vi "JocAcabatEntregableAmbSubVis.vi"() -> ()   [LabVIEW 2023]
uses:
  <vilib>/MakerHub/LINX/Private/Local IO/LinxAnalogRead.vi
  <vilib>/MakerHub/LINX/Public/Utilities/Check Channel.vi
  <vilib>/MakerHub/LINX/Private/Utilties/Generate Error.vi
  <vilib>/MakerHub/LINX/Private/Device/Peripheral/Analog/Analog Read.vi
  <vilib>/MakerHub/LINX/Public/Utilities/Open Serial.vi
  <vilib>/MakerHub/LINX/LMH-LINX.lvlib
panel:
  out "?":string
  out "?":string="Benvingut a la jungla! El teu objectiu és sobreviure! Per aconseguir-ho, has de caçar les preses (punts verds) i fugir dels depredadors (punts vermells). Alerta, a mida que vagis avançant en el joc, aniràn apreixent més preses i depredadors. Per sort, si t'estàs a punt de quedar sense vides, apareixerà un quadrat groc, si l'atrapes, et proporcionarà una vida extra. També has de tenir en compte que tens 40 s per atrapar les preses, si tardes més, et moriràs de gana... Abans que passi però, apareixerà un diamant groc. Atrapa'l i tindràs una mica més de temps per caçar. Bona sort! "
  out "Nivell:":i32
  in  "base path":path
  in  "Serial Port":refnum<visa-resource-name>="N/A"
  out "Tablero":cluster{dbl[], dbl[]}[](graph)
  out "Vides":i32
  out "Preses capturades":i32
  out "Temps sense \nmenjar (ms)":u32
  in  "?":bool
  out "ms totals":u32
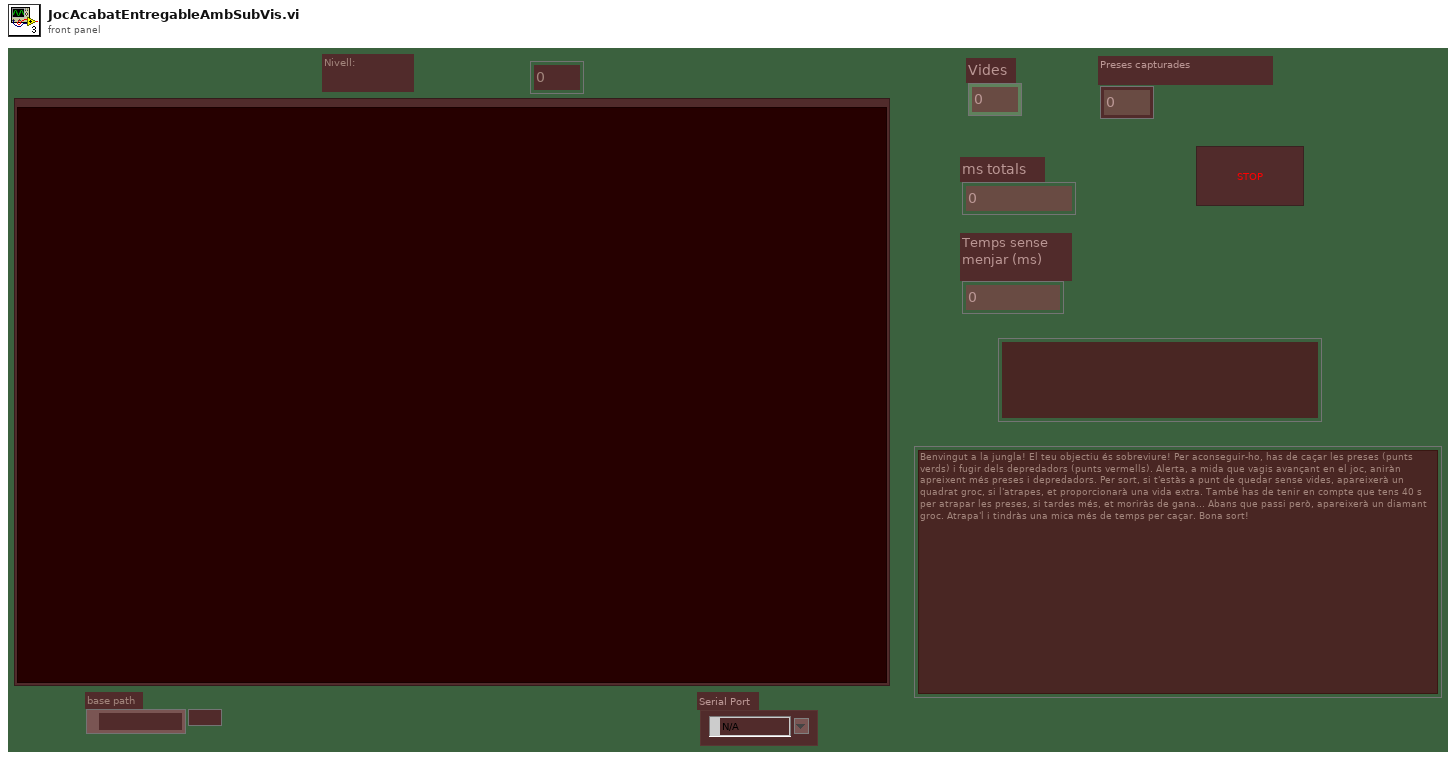
[diagram p1: front panel]
types:
  T1 = enum16{"open", "replace", "create", "open or create", "replace or create", "replace or create with confirmation"}
  T2 = typedef "LMH-LINX.lvlib/LINX Ref.ctl" = cluster{"IO":T3, "Interface":T4, "LINX Device Config":T5}
  T3 = typedef "LMH-LINX.lvlib/Platform.ctl" = enum16{"Remote", "Local"}
  T4 = typedef "LMH-LINX.lvlib/Interface.ctl" = enum16{"Serial", "TCP"}
  T5 = typedef "LMH-LINX.lvlib/Device.lvlib/LINX Device Config.ctl" = cluster{"Interface":T4, "COM Port":refnum<visa-resource-name>, "TCP Configuration":T6, "Device Family":u8, "Device ID":u8, "Device Name":string, "TCP Ref":refnum<k5>, "Channels":T7}
  T6 = typedef "LMH-LINX.lvlib/Device.lvlib/TCP Config.ctl" = cluster{"IP Address":string, "Port":u16}
  T7 = typedef "LMH-LINX.lvlib/Channels.ctl" = cluster{"DI":u8[], "DO":u8[], "AI":u8[], "AO":u8[], "PWM":u8[], "QE":u8[], "UART":u8[], "I2C 2":u8[], "SPI":u8[], "CAN":u8[], "Servo":u8[], "AI Ref (V)":dbl, "AI Resolution (Bits)":u8, "AO Ref (V)":dbl, "AO Resolution (Bits)":u8}
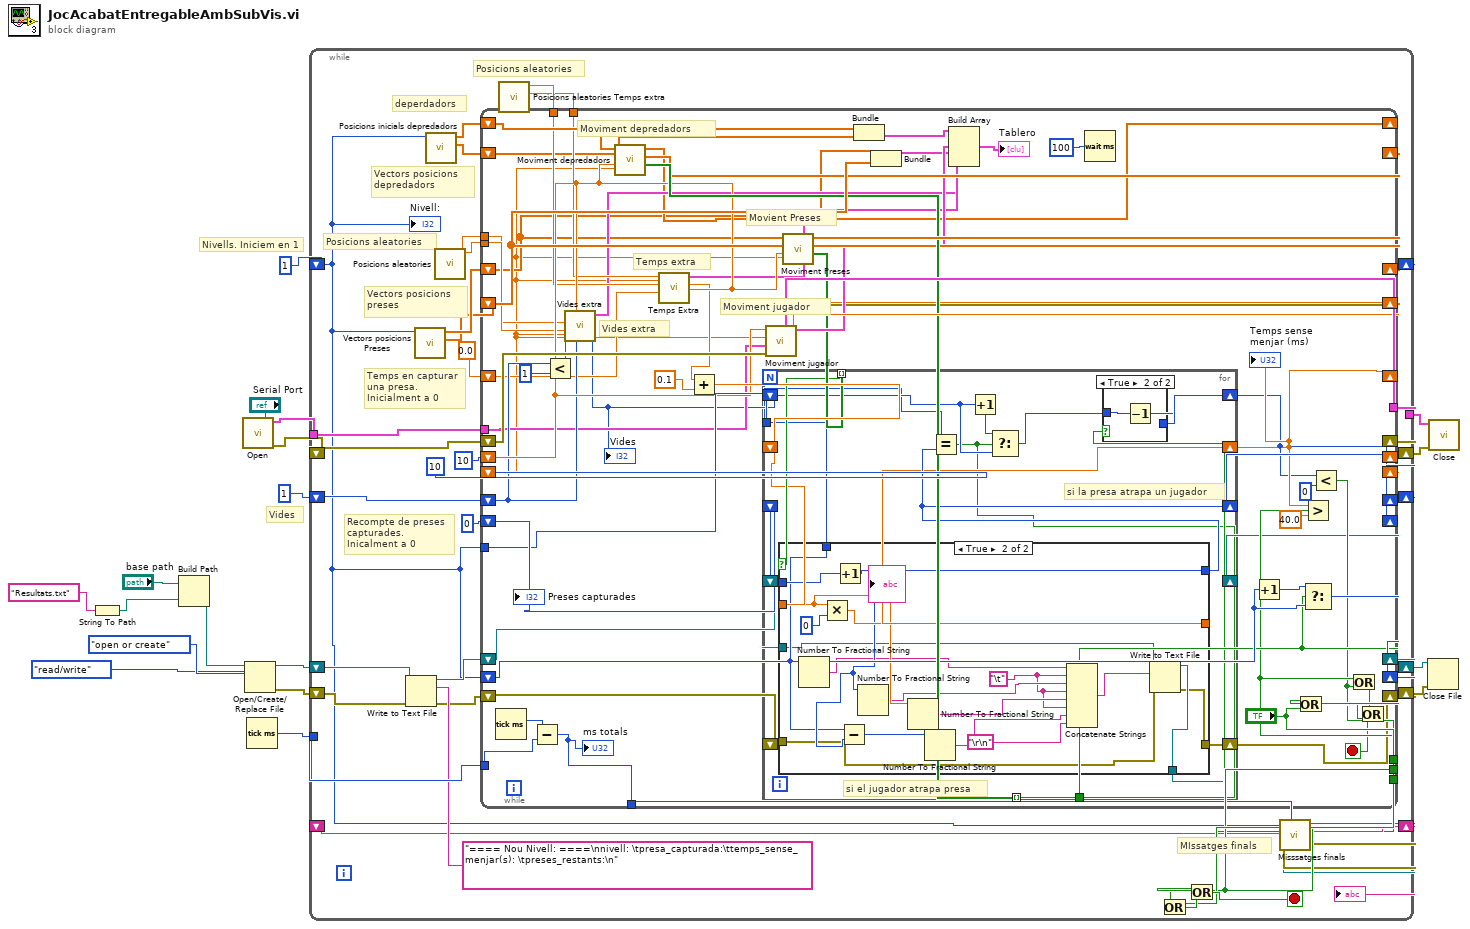
[diagram p0: block diagram]
diagram:
  # "Nivells. Iniciem en 1"
  # "Vides"
  n1 = String To Path(string="Resultats.txt") -> (path=w4:path)
  n2 = Build Path(base path="base path", name or relative path=w4) -> (appended path=w7:path)
  n3 = call-poly <vilib>:"Open.vi"("Serial Port"="Serial Port") -> ("Error Out"=w12:errorcluster, "LINX Resource"=w13:T2)  [unwired: 8 in, 1 out]
  n4 = Open/Create/Replace File(file path (use dialog)=w7, operation (0:open)=T1."open or create", access (0:read/write)=enum16{"read/write", "read-only", "write-only"}."read/write") -> (refnum out=w1:refnum<file>, error out=w8:errorcluster)  [unwired: 3 in, 1 out]
  n5 = Tick Count (ms)() -> (millisecond timer value=w17:u32)
  n6 = while {
    shift-right: [w51] -> _
    shift-left: 1 -> [w24]
    tunnel: w17 -> [w42]
    shift-right: [w48] -> _
    shift-left: 1 -> [w49]
    tunnel: [w46] -> w14
    tunnel: w13 -> [w45]
    shift-right: [w47] -> w15
    shift-left: w12 -> [w43]
    shift-right: [w28] -> w3
    shift-left: w8 -> [w31]
    shift-right: [w27] -> w2
    shift-left: w1 -> [w32]
    shift-right: [w25] -> _
    shift-left: _ -> [w26]
    stop <- w36 stop-if-true
    # "MIssatges finals"
    # "Temps en capturar \nuna presa. \nInicialment a 0"
    # "Recompte de preses \ncapturades. \nInicalment a 0"
    # "Vectors posicions \npreses"
    # "Vectors posicions \ndepredadors"
    # "Posicions aleatories"
    # "Posicions aleatories"
    # "deperdadors"
    n7 = Write to Text File(file (use dialog)=w32, text="==== Nou Nivell: ====\nnivell: \tpresa_capturada:\ttemps_sense_menjar(s): \tpreses_restants:\n", error in=w31) -> (refnum out=w33:refnum<file>, error out=w30:errorcluster)  [unwired: 1 in, 1 out]
    n8 = call "Vectors posicions Preses.vi"("Numeric"=w24) -> ("Array"=w53:dbl[], "Array 2"=w54:dbl[])  [unwired: 9 in]
    n9 = call "Posicions inicials depredadors.vi"("Numeric"=w24) -> ("Array"=w55:dbl[], "Array 2"=w56:dbl[])  [unwired: 9 in]
    n10 = call "Posicions aleatories.vi"() -> ("Numeric"=w38:dbl, "Numeric 2"=w39:dbl)  [unwired: 10 in]
    n11 = call "Posicions aleatories Temps extra.vi"() -> ("Numeric"=w20:dbl, "Numeric 2"=w40:dbl)  [unwired: 10 in]
    n12 = while {
      shift-right: [w69] -> _
      shift-left: w56 -> [w90]
      shift-right: [w105] -> _
      shift-left: w55 -> [w70]
      shift-right: [w112] -> _
      shift-left: w54 -> [w67]
      shift-right: [w107] -> _
      shift-left: w53 -> [w113]
      shift-right: [w61] -> _
      shift-left: 10 -> [w87]
      shift-right: [w114] -> _
      shift-left: 10 -> [w63]
      shift-right: [w64] -> w47
      shift-left: w43 -> [w116]
      tunnel: [w115] -> w46
      shift-right: [w57] -> w48
      shift-left: w49 -> [w86]
      shift-right: [w109] -> _
      shift-left: 0 -> [w111]
      tunnel: w24 -> [w106]
      tunnel: [w96] -> w35
      shift-right: [w103] -> w51
      shift-left: w24 -> [w104]
      tunnel: w45 -> [w66]
      tunnel: ["?"] -> w21
      tunnel: w42 -> [w100]
      shift-right: [w58] -> _
      shift-left: 0.0 -> [w85]
      tunnel: [w92] -> w34
      tunnel: w40 -> [w81]
      tunnel: w20 -> [w80]
      tunnel: w39 -> [w79]
      tunnel: w38 -> [w78]
      shift-right: [w76] -> w22
      shift-left: w33 -> [w71]
      tunnel: [w75] -> w19
      shift-right: [w73] -> w29
      shift-left: w30 -> [w74]
      stop <- w59 stop-if-true
      # "Moviment jugador"
      # "Moviment depredadors"
      # "Vides extra"
      # "Temps extra"
      # "Movient Preses"
      n13 = Tick Count (ms)() -> (millisecond timer value=w101:u32)
      n14 = Subtract(x=w101, y=w100) -> (x-y=w75:u32)
      "ms totals" <- w75
      n15 = Less?(x=w86, y=1) -> (x < y?=w88:bool)
      n16 = call "Vides extra.vi"("Numeric 5"=w63, "Numeric 6"=w87, "Numeric 4"=w86, "Numeric 2"=w79, "Numeric"=w78, "Boolean"=w88) -> ("Numeric 3"=w60:i32, "Cluster"=w72:cluster{dbl[], dbl[]})  [unwired: 4 in]
      "Vides" <- w60
      n17 = call "Moviment depredadors.vi"("Numeric"=w63, "Numeric 2"=w87, "Array"=w70, "Array 2"=w90) -> ("Array 4"=w110:bool[], "Array 3"=w105:dbl[], "Array 5"=w69:dbl[])  [unwired: 5 in]
      n18 = call "Temps Extra.vi"("Numeric 6"=w87, "Numeric 5"=w63, "Numeric 4"=w85, "Numeric 2"=w81, "Numeric"=w80) -> ("Numeric 3"=w84:dbl, "Cluster"=w83:cluster{dbl[], dbl[]})  [unwired: 5 in]
      n19 = Add(x=w84, y=0.1) -> (x+y=w98:dbl)
      n20 = call "Moviment jugador.vi"("error in (no error)"=w116, "LINX Resource in"=w66, "Numeric"=w63, "Numeric 2"=w87) -> ("error out"=w64:errorcluster, "Numeric 3"=w114:dbl, "Numeric 4"=w61:dbl, "Cluster"=w89:cluster{dbl[], dbl[]}, "LINX Resource out"=w115:T2)  [unwired: 3 in]
      n21 = call "Moviment Preses.vi"("Numeric"=w63, "Numeric 2"=w87, "Array 5"=w113, "Array 3"=w67) -> ("Array"=w77:bool[], "Array 2"=w107:dbl[], "Array 4"=w112:dbl[])  [unwired: 5 in]
      n22 = for {
        tunnel: w77 -> [w131] mode=indexing
        shift-right: [w126] -> w109
        shift-left: w111 -> [w130]
        tunnel: w106 -> [w121]
        shift-right: [w127] -> w57
        shift-left: w60 -> [w129]
        tunnel: w110 -> [w128] mode=indexing
        shift-right: [w125] -> w58
        shift-left: w98 -> [w124]
        tunnel: [w123] -> w97
        shift-right: [w118] -> w73
        shift-left: w74 -> [w119]
        shift-right: [w120] -> w76
        shift-left: w71 -> [w122]
        # "si la presa atrapa un jugador"
        # "si el jugador atrapa presa"
        n23 = case shown="True" w131 {
          tunnel: [w140 w154] -> w126
          tunnel: w130 -> [w140 w158]
          tunnel: w124 -> [w139 w155]
          tunnel: [w139 w157] -> w125
          tunnel: w122 -> [w138 w146]
          tunnel: w121 -> [_ w148]
          tunnel: [w138 w152] -> w120
          tunnel: w119 -> [w137 w151]
          tunnel: [w137 w150] -> w118
          frame False {
          }
          frame True {
            w143 = "\t"
            n24 = Number To Fractional String(number=w148) -> (F-format string=w147:string)  [unwired: 3 in]
            n25 = Multiply(x=w155, y=0) -> (x*y=w157:dbl)
            n26 = Increment(x=w158) -> (x+1=w154:i32)
            n27 = Subtract(x=w148, y=w154) -> (x-y=w153:i32)
            n28 = Number To Fractional String(number=w154) -> (F-format string=w145:string)  [unwired: 3 in]
            n29 = Number To Fractional String(number=w155) -> (F-format string=w144:string)  [unwired: 3 in]
            n30 = Number To Fractional String(number=w153) -> (F-format string=w142:string)  [unwired: 3 in]
            n31 = Concatenate Strings(w147, w143, w145, w143, w144, w143, w142, "\r\n") -> (w149:string)
            n32 = Write to Text File(file (use dialog)=w146, text=w149, error in=w151) -> (refnum out=w152:refnum<file>, error out=w150:errorcluster)  [unwired: 1 in, 1 out]
          }
        }
        n33 = Equal?(x=w121, y=w126) -> (x = y?=w123:bool)
        n34 = Increment(x=w129) -> (x+1=w133:i32)
        n35 = Select(t=w133, s=w123, f=w129) -> (s? t:f=w132:i32)
        n36 = case shown="True" w128 {
          tunnel: w132 -> [w134 w136]
          tunnel: [w134 w135] -> w127
          frame False {
          }
          frame True {
            n37 = Decrement(x=w136) -> (x-1=w135:i32)
          }
        }
      }
      "Temps sense \nmenjar (ms)" <- w58
      n38 = Bundle("Array 5"=w90, "Array 3"=w70) -> (w65:cluster{"Array 5":dbl[], "Array 3":dbl[]})  [unwired: 1 in]
      n39 = Bundle("Array 4"=w67, "Array 2"=w113) -> (w68:cluster{"Array 4":dbl[], "Array 2":dbl[]})  [unwired: 1 in]
      n40 = Build Array(w65, w68, w89, w72, w83) -> (→"Tablero":cluster{"Array 4":dbl[], "Array 2":dbl[]}[])
      n41 = Wait (ms)(milliseconds to wait=u32 100) -> ()  [unwired: 1 out]
      n42 = Increment(x=w104) -> (x+1=w62:i32)
      n43 = Or(x=w97, y="?") -> (x .or. y?=w93:bool)
      n44 = Greater?(x=w58, y=40.0) -> (0:w96:bool)
      n45 = Select(t=w62, s=w97, f=w104) -> (s? t:f=w103:i32)
      n46 = Less?(x=w57, y=0) -> (x < y?=w92:bool)
      n47 = Or(x=w96, y=w92) -> (x .or. y?=w94:bool)
      n48 = Or(x=w94, y=w93) -> (x .or. y?=w59:bool)
      "Preses capturades" <- w111
    }
    n49 = Or(x=w35, y=w21) -> (x .or. y?=w41:bool)
    n50 = Or(x=w34, y=w41) -> (x .or. y?=w36:bool)
    n51 = call "Misssatges finals.vi"("result string in"=w26, "Boolean"=w34, "Numeric 2"=w19, "Boolean 2"=w35, "error in (no error)"=w29, "Numeric"=w24, "Boolean 3"=w21, "Byte Stream File in"=w22) -> ("error out"=w28:errorcluster, "result string out"=w25:string, "Byte Stream File out"=w27:refnum<file>)  [unwired: 1 in]
    "?" <- w25
    "Nivell:" <- w24
  }
  n52 = Close File(refnum=w2, error in=w3) -> ()  [unwired: 2 out]
  n53 = call <vilib>:"Close.vi"("Error In"=w15, "LINX Resource"=w14) -> ()  [unwired: 9 in, 1 out]
